vi "Manual_Test.vi"(9 "data":variant, 10 "station":string, 11 "URL":string) -> (3 "ok?":bool)   [LabVIEW 2012]
uses:
  Globals/Global.vi
  read_Array.vi
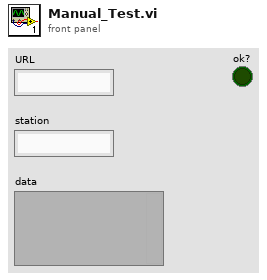
[diagram p1: front panel]
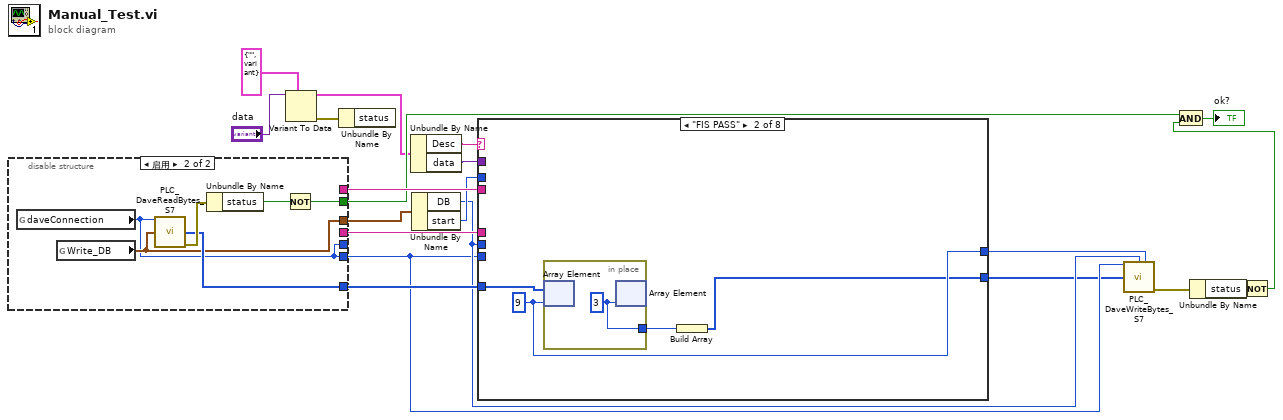
[diagram p0: block diagram]
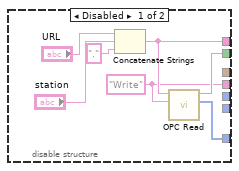
[diagram p2: hidden frame]
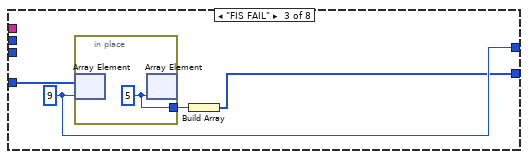
[diagram p4: hidden frame]
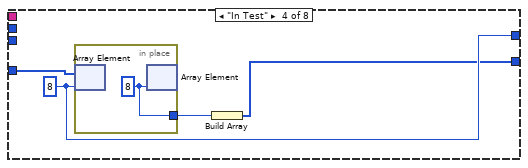
[diagram p5: hidden frame]
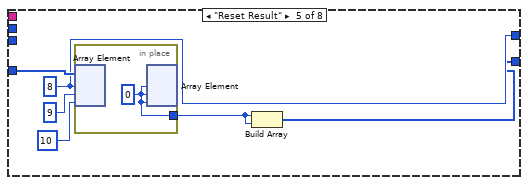
[diagram p6: hidden frame]
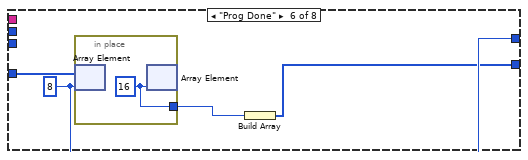
[diagram p7: hidden frame]
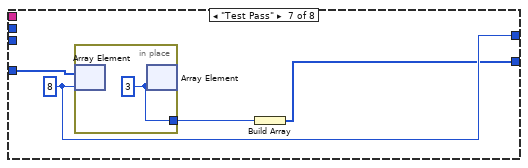
[diagram p8: hidden frame]
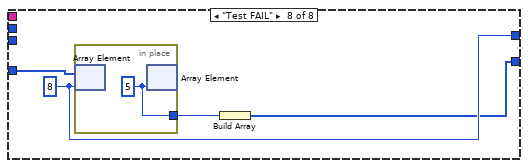
[diagram p9: hidden frame]
diagram:
  n1 = disable-structure shown="启用" {
    disable-tunnel: [w26 w30] -> w18
    disable-tunnel: [w23 _] -> w17
    disable-tunnel: [w22 w31] -> w16
    disable-tunnel: [w21 _] -> w10
    disable-tunnel: [_ w28] -> w4
    disable-tunnel: [_ w29] -> w9
    disable-tunnel: [_ w28] -> _
    frame Disabled {
      w21 = "Write" ("Address")
      n2 = Concatenate Strings("URL", "station", "." ("string")) -> (w23:string)
      n3 = call-poly "OPC Read.vi"("Address"=w21, "URL"=w23) -> ("Value"=w26:u8[], "ok?"=w22:bool)  [unwired: 7 in, 1 out]
    }
    frame Enabled {
      n4 = global read "Global.vi" "daveConnection"() -> (w28:i64)
      n5 = global read "Global.vi" "Write_DB"() -> (w29:cluster{"DB":i32, "start":i32, "len":i32})
      n6 = call "PLC_DaveReadBytes_S7.vi"("daveConnection in"=w28, "地址"=w29) -> ("read Buffer"=w30:u8[], "error out"=w32:errorcluster)  [unwired: 10 in, 2 out]
      n7 = Unbundle By Name(w32) -> ("status"=w33:bool)
      n8 = Not(x=w33) -> (.not. x?=w31:bool)
    }
  }
  n9 = Variant To Data(type=cluster{"Desc":string, "data":variant} {"Desc"="", "data"=variant}, Variant="data") -> (data=w13:cluster{"Desc":string, "data":variant}, error out=w20:errorcluster)  [unwired: 1 in]
  n10 = Unbundle By Name(w20) -> ()  [unwired: 1 out]
  n11 = Unbundle By Name(w13) -> ("Desc"=w12:string, "data"=w11:variant)
  n12 = Unbundle By Name(w9) -> ("DB"=w5:i32, "start"=w8:i32)
  n13 = case shown="\"FIS PASS\"" w12 {
    tunnel: w17 -> [_ _ _ _ _ _ _ _]
    tunnel: w18 -> [_ w37 w42 w47 w54 w59 w64 w69]
    tunnel: w11 -> [_ _ _ _ _ _ _ _]
    tunnel: w10 -> [_ _ _ _ _ _ _ _]
    tunnel: w4 -> [_ _ _ _ _ _ _ _]
    tunnel: w5 -> [_ _ _ _ _ _ _ _]
    tunnel: w8 -> [_ _ _ _ _ _ _ _]
    tunnel: [_ w36 w41 w46 w51 w58 w63 w68] -> w3
    tunnel: [_ w34 w39 w44 w49 w56 w61 w66] -> w1
    frame Default {
    }
    frame "FIS PASS" {
      w36 = 9
      n14 = in-place {
        in-place-border: [w38] -> w35
        w38 = u8 3 ("element")
        n15 = in-place-array #1(w37, w36) -> ()  [unwired: 1 out]
        n16 = in-place-array #1(w38) -> ()  [unwired: 2 out]
      }
      n17 = Build Array(w35) -> (w34:u8[])
    }
    frame "FIS FAIL" {
      w41 = 9
      n18 = in-place {
        in-place-border: [w43] -> w40
        w43 = u8 5 ("element")
        n19 = in-place-array #2(w42, w41) -> ()  [unwired: 1 out]
        n20 = in-place-array #2(w43) -> ()  [unwired: 2 out]
      }
      n21 = Build Array(w40) -> (w39:u8[])
    }
    frame "In Test" {
      w46 = 8
      n22 = in-place {
        in-place-border: [w48] -> w45
        w48 = u8 8 ("element")
        n23 = in-place-array #3(w47, w46) -> ()  [unwired: 1 out]
        n24 = in-place-array #3(w48) -> ()  [unwired: 2 out]
      }
      n25 = Build Array(w45) -> (w44:u8[])
    }
    frame "Reset Result" {
      w51 = 8
      n26 = in-place {
        in-place-border: [w55] -> w50
        w55 = u8 0 ("element")
        n27 = in-place-array #4(w54, w51, 9, 10) -> ()  [unwired: 3 out]
        n28 = in-place-array #4(w55, w55, w55) -> ()  [unwired: 4 out]
      }
      n29 = Build Array(w50, w50) -> (w49:u8[])
    }
    frame "Prog Done" {
      w58 = 8
      n30 = in-place {
        in-place-border: [w60] -> w57
        w60 = u8 16 ("element")
        n31 = in-place-array #5(w59, w58) -> ()  [unwired: 1 out]
        n32 = in-place-array #5(w60) -> ()  [unwired: 2 out]
      }
      n33 = Build Array(w57) -> (w56:u8[])
    }
    frame "Test Pass" {
      w63 = 8
      n34 = in-place {
        in-place-border: [w65] -> w62
        w65 = u8 3 ("element")
        n35 = in-place-array #6(w64, w63) -> ()  [unwired: 1 out]
        n36 = in-place-array #6(w65) -> ()  [unwired: 2 out]
      }
      n37 = Build Array(w62) -> (w61:u8[])
    }
    frame "Test FAIL" {
      w68 = 8
      n38 = in-place {
        in-place-border: [w70] -> w67
        w70 = u8 5 ("element")
        n39 = in-place-array #7(w69, w68) -> ()  [unwired: 1 out]
        n40 = in-place-array #7(w70) -> ()  [unwired: 2 out]
      }
      n41 = Build Array(w67) -> (w66:u8[])
    }
  }
  n42 = call "PLC_DaveWriteBytes_S7.vi"("daveConnectionIN"=w4, "DB"=w5, "start"=w3, "Buffer"=w1) -> ("error out"=w6:errorcluster)  [unwired: 9 in, 2 out]
  n43 = Unbundle By Name(w6) -> ("status"=w7:bool)
  n44 = Not(x=w7) -> (.not. x?=w2:bool)
  n45 = And(x=w16, y=w2) -> (x .and. y?=→"ok?":bool)
